vi "Add Hero Image.vi"(8 "error in (no error)":errorcluster, 9 "alternateText":string, 10 "Image":path, 11 "reference":refnum<k24>) -> (0 "error out":errorcluster, 3 "reference out":refnum<k24>)   [LabVIEW 2020, in "ToastNotification.lvlib" / "Toast Native.lvlib"]
doc: "Converts the local image path to a System.Uri and adds it as a hero image to the supplied ToastContentBuilder. Releases the temporary URI reference after the call, including on error. The caller owns the builder reference."
uses:
  Toast Native.lvlib
  C:/Users/loicw/Documents/LabVIEW/ToastNotifications/Sources/bins/Microsoft.Toolkit.Uwp.Notifications.dll
  bins/Microsoft.Toolkit.Uwp.Notifications.dll
  Reflection DotNet/Reflection DotNet.lvlib
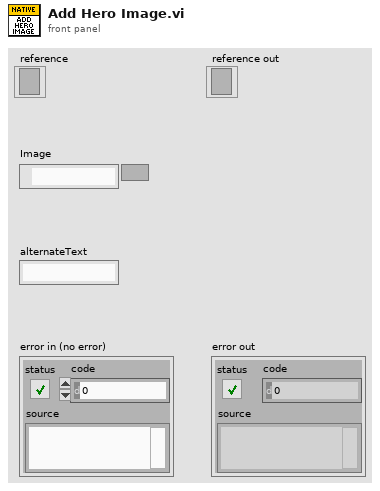
[diagram p1: front panel]
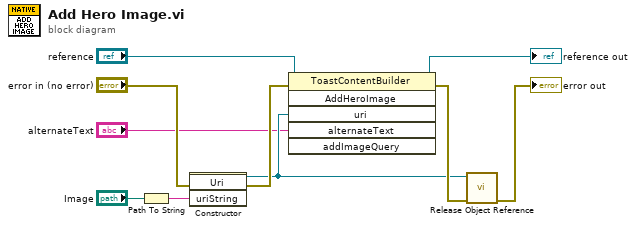
[diagram p0: block diagram]
diagram:
  n1 = Path To String(path="Image") -> (string=w7:string)
  n2 = constructor class="Uri"(error in="error in (no error)", "uriString"=w7) -> (reference out=w2:refnum<k24>, error out=w5:errorcluster)  [unwired: 2 in, 2 out]
  n3 = invoke class="ToastContentBuilder" method="AddHeroImage"(reference="reference", error in=w5, "uri"=w2, "alternateText"="alternateText") -> (reference out=→"reference out":refnum<k24>, error out=w4:errorcluster)  [unwired: 2 in, 4 out]
  n4 = call "Release Object Reference.vi"("error in"=w4, "object"=w2) -> ("error out"=→"error out":errorcluster)  [unwired: 9 in]
